vi "Modify Item Owner.vi"(8 "error in (no error)":errorcluster, 9 "New Parent Fully Qualified Name":string, 10 "UniqueName Object":refnum<class "UniqueName.lvclass">, 11 "Registry in":refnum<data-value>) -> (0 "error out":errorcluster, 1 "Modified":bool, 2 "UniqueName Object out":refnum<class "UniqueName.lvclass">, 3 "Registry":refnum<data-value>)   [LabVIEW 2013, in "UniqueName.lvlib" / "NameRegistry.lvclass"]
uses:
  NameRegistry.lvclass
  UniqueNameClass/UniqueName.lvclass
  UniquenessCriteria/UniquenessCriteria.lvclass
  UniqueNameClass/Key.ctl
  StringIncrement/StringIncrement.lvclass
  RandomStringGenerator/RandomStringGenerator.lvclass
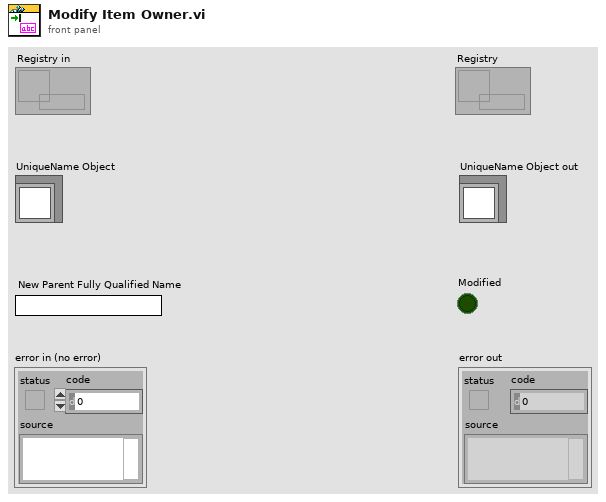
[diagram p1: front panel]
types:
  T1 = typedef "UniqueName.lvlib/UniqueName.lvclass/Key.ctl" = enum16{"Fully Qualified Name", "Unique Name", "Given Name", "Parent Fully Qualified Name", "UUID"}
  T2 = typedef "UniqueName.lvlib/UniquenessCriteria.lvclass/Criteria.ctl" = enum16{"Globally-Unique Fully Qualified Name", "Globally-Unique Name", "Universal Unique Identifier"}
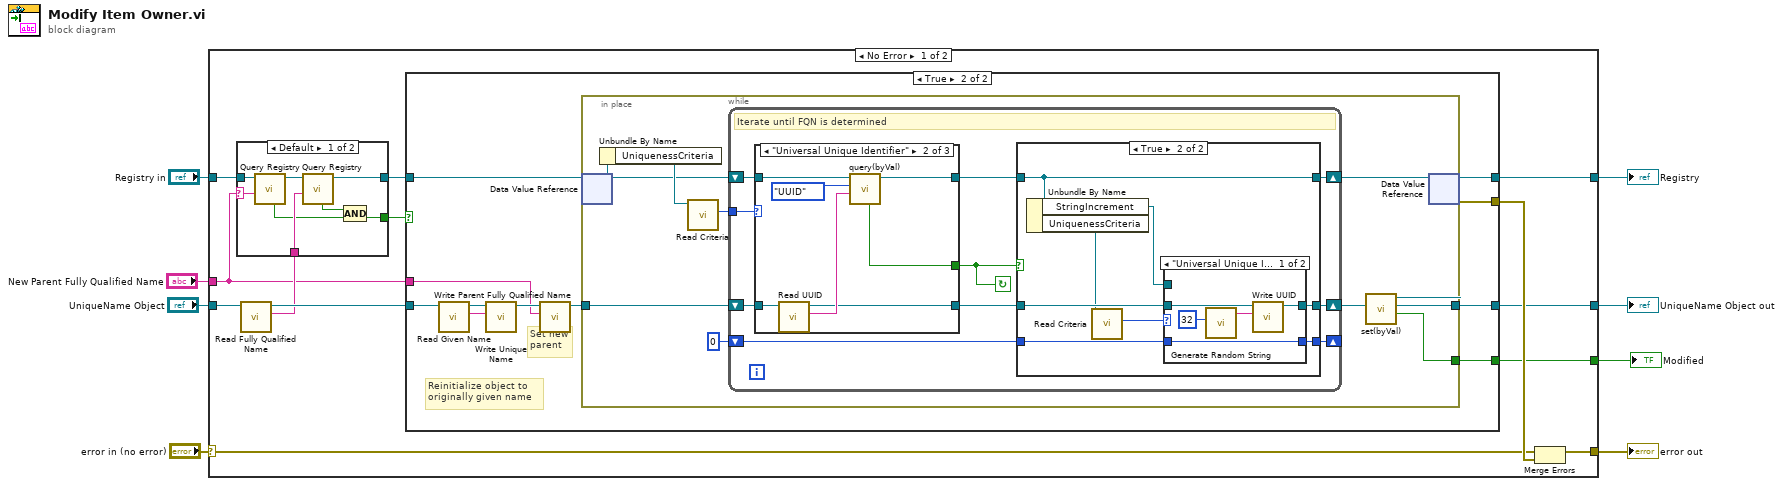
[diagram p0: block diagram]
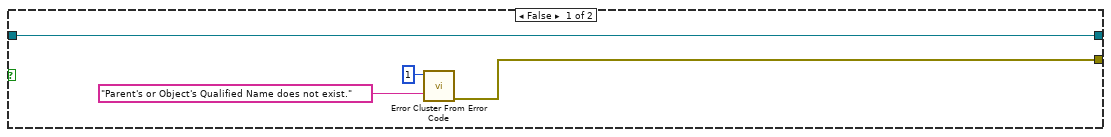
[diagram p2: hidden frame]
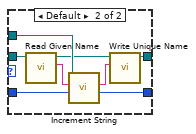
[diagram p4: hidden frame]
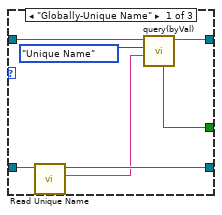
[diagram p5: hidden frame]
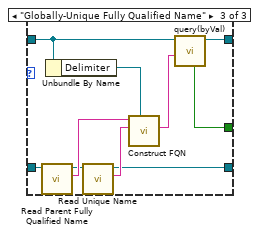
[diagram p6: hidden frame]
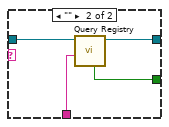
[diagram p7: hidden frame]
diagram:
  n1 = case shown="No Error" "error in (no error)" {
    selector: "error in (no error)" -> [w19 w118]
    tunnel: "Registry in" -> [w17 w119]
    tunnel: [w21 w119] -> w7
    tunnel: [w18 w118] -> w5
    tunnel: "New Parent Fully Qualified Name" -> [w10 _]
    tunnel: [w14 w117] -> w3
    tunnel: "UniqueName Object" -> [w13 w117]
    tunnel: [w9 _] -> w1
    frame No Error {
      n2 = call "Read Fully Qualified Name.vi"("UniqueName in"=w13) -> ("Fully Qualified Name"=w11:string, "UniqueName out"=w12:refnum<class "UniqueName.lvclass">)  [unwired: 9 in]
      n3 = case shown="Default" w10 {
        selector: w10 -> [w111 _]
        tunnel: w17 -> [w112 w114]
        tunnel: [w109 w116] -> w16
        tunnel: [w106 w113] -> w15
        tunnel: w11 -> [w108 w115]
        frame Default {
          n4 = call "Query Registry.vi"("Search string"=w111, "Registry in"=w112) -> ("Registry"=w110:refnum<data-value>, "found?"=w107:bool)  [unwired: 5 in, 3 out]
          n5 = call "Query Registry.vi"("Search string"=w108, "Registry in"=w110) -> ("Registry"=w109:refnum<data-value>, "found?"=w105:bool)  [unwired: 5 in, 3 out]
          n6 = Compound Arithmetic op=AND(w105, w107) -> (w106:bool)
        }
        frame "" {
          n7 = call "Query Registry.vi"("Search string"=w115, "Registry in"=w114) -> ("Registry"=w116:refnum<data-value>, "found?"=w113:bool)  [unwired: 5 in, 3 out]
        }
      }
      n8 = case shown="True" w15 {
        tunnel: [w25 w36] -> w21
        tunnel: [w23 w35] -> w20
        tunnel: w16 -> [w25 w32]
        tunnel: w10 -> [_ w33]
        tunnel: [_ w30] -> w14
        tunnel: w12 -> [_ w29]
        tunnel: [_ w26] -> w9
        frame False {
          n9 = call <vilib>:"Error Cluster From Error Code.vi"("error message (\"\")"="Parent's or Object's Qualified Name does not exist." ("error message (\"\")"), "error code (0)"=1) -> ("error out"=w23:errorcluster)  [unwired: 7 in]
        }
        frame True {
          # "Set new\nparent"
          # "Reinitialize object to\noriginally given name"
          n10 = call "Read Given Name.vi"("UniqueName in"=w29) -> ("Given Name"=w28:string, "UniqueName out"=w27:refnum<class "UniqueName.lvclass">)  [unwired: 9 in]
          n11 = call "Write Unique Name.vi"("Unique Name"=w28, "UniqueName in"=w27) -> ("UniqueName out"=w34:refnum<class "UniqueName.lvclass">)  [unwired: 9 in]
          n12 = call "Write Parent Fully Qualified Name.vi"("Parent Fully Qualified Name"=w33, "UniqueName in"=w34) -> ("UniqueName out"=w31:refnum<class "UniqueName.lvclass">)  [unwired: 9 in]
          n13 = in-place {
            in-place-border: w31 -> [w44]
            in-place-border: [w41] -> w30
            in-place-border: [w38] -> w26
            n14 = in-place-dvr #1(w32) -> (w43:refnum<class "NameRegistry.lvclass">)  [unwired: 1 out]
            n15 = Unbundle By Name(w43) -> ("UniquenessCriteria"=w46:refnum<class "UniquenessCriteria.lvclass">)
            n16 = call "Read Criteria.vi"("UniquenessCriteria in"=w46) -> ("Criteria"=w45:T2)  [unwired: 9 in, 1 out]
            n17 = while {
              tunnel: w45 -> [w56]
              shift-right: [w54] -> w42
              shift-left: w44 -> [w53]
              shift-right: [w49] -> w40
              shift-left: w43 -> [w51]
              shift-right: [w48] -> _
              shift-left: u32 0 ("Incremented Numeric") -> [w47]
              stop <- w52 continue-if-true
              # "Iterate until FQN is determined"
              n18 = case shown="\"Universal Unique Identifier\"" w56 {
                tunnel: [w84 w93 w98] -> w52
                tunnel: w53 -> [w87 w90 w102]
                tunnel: [w86 w88 w100] -> w55
                tunnel: w51 -> [w85 w94 w96]
                tunnel: [w81 w91 w97] -> w50
                frame "Globally-Unique Name" {
                  n19 = call "Read Unique Name.vi"("UniqueName in"=w87) -> ("Unique Name"=w82:string, "UniqueName out"=w86:refnum<class "UniqueName.lvclass">)  [unwired: 9 in]
                  n20 = call "query(byVal).vi"("Search string"=w82, "Search Key (FQN)"=Key."Unique Name" ("Key (FQN)"), "Instance"=w85) -> ("Instance"=w81:refnum<class "NameRegistry.lvclass">, "found?"=w84:bool)  [unwired: 5 in, 2 out]
                }
                frame "Universal Unique Identifier" {
                  n21 = call "Read UUID.vi"("UniqueName in"=w90) -> ("UUID"=w89:string, "UniqueName out"=w88:refnum<class "UniqueName.lvclass">)  [unwired: 9 in]
                  n22 = call "query(byVal).vi"("Search string"=w89, "Search Key (FQN)"=Key."UUID" ("Key (FQN)"), "Instance"=w94) -> ("Instance"=w91:refnum<class "NameRegistry.lvclass">, "found?"=w93:bool)  [unwired: 5 in, 2 out]
                }
                frame "Globally-Unique Fully Qualified Name" {
                  n23 = call "Read Parent Fully Qualified Name.vi"("UniqueName in"=w102) -> ("Parent Fully Qualified Name"=w104:string, "UniqueName out"=w101:refnum<class "UniqueName.lvclass">)  [unwired: 9 in]
                  n24 = Unbundle By Name(w96) -> ("Delimiter"=w95:refnum<class "Delimiter.lvclass">)
                  n25 = call "Read Unique Name.vi"("UniqueName in"=w101) -> ("Unique Name"=w103:string, "UniqueName out"=w100:refnum<class "UniqueName.lvclass">)  [unwired: 9 in]
                  n26 = call "Construct FQN.vi"("Delimiter"=w95, "Name"=w103, "Parent FQN"=w104) -> ("FQN"=w99:string)  [unwired: 8 in]
                  n27 = call "query(byVal).vi"("Search string"=w99, "Instance"=w96) -> ("Instance"=w97:refnum<class "NameRegistry.lvclass">, "found?"=w98:bool)  [unwired: 6 in, 2 out]
                }
              }
              n28 = case shown="True" w52 {
                tunnel: w55 -> [w59 w64]
                tunnel: [w59 w67] -> w54
                tunnel: w50 -> [w58 w66]
                tunnel: [w58 w66] -> w49
                tunnel: [w57 w63] -> w48
                tunnel: w47 -> [w57 w62]
                frame False {
                  # "Name already unique"
                }
                frame True {
                  n29 = Unbundle By Name(w66) -> ("StringIncrement"=w65:refnum<class "StringIncrement.lvclass">, "UniquenessCriteria"=w61:refnum<class "UniquenessCriteria.lvclass">)
                  n30 = call "Read Criteria.vi"("UniquenessCriteria in"=w61) -> ("Criteria"=w60:T2)  [unwired: 9 in, 1 out]
                  n31 = case shown="\"Universal Unique Identifier\"" w60 {
                    tunnel: [w71 w80] -> w67
                    tunnel: w65 -> [_ w78]
                    tunnel: w64 -> [w70 w77]
                    tunnel: [w72 w74] -> w63
                    tunnel: w62 -> [w72 w73]
                    frame "Universal Unique Identifier" {
                      n32 = call "Generate Random String.vi"("String Length (32)"=u32 32) -> ("Random String"=w69:string)  [unwired: 10 in]
                      n33 = call "Write UUID.vi"("UUID"=w69, "UniqueName in"=w70) -> ("UniqueName out"=w71:refnum<class "UniqueName.lvclass">)  [unwired: 9 in]
                    }
                    frame Default {
                      n34 = call "Read Given Name.vi"("UniqueName in"=w77) -> ("Given Name"=w76:string, "UniqueName out"=w75:refnum<class "UniqueName.lvclass">)  [unwired: 9 in]
                      n35 = call "Increment String.vi"("Numeric"=w73, "Input String"=w76, "StringIncrement"=w78) -> ("Incremented Numeric"=w74:u32, "Incremented String"=w79:string)  [unwired: 7 in]
                      n36 = call "Write Unique Name.vi"("Unique Name"=w79, "UniqueName in"=w75) -> ("UniqueName out"=w80:refnum<class "UniqueName.lvclass">)  [unwired: 9 in]
                    }
                  }
                }
              }
            }
            n37 = call "set(byVal).vi"("UniqueName in"=w42, "NameRegistry in"=w40) -> ("Replaced?"=w38:bool, "UniqueName out"=w41:refnum<class "UniqueName.lvclass">, "NameRegistry out"=w39:refnum<class "NameRegistry.lvclass">)  [unwired: 7 in]
            n38 = in-place-dvr #1(w39) -> (w36:refnum<data-value>, w35:errorcluster)
          }
        }
      }
      n39 = Merge Errors(w19, w20) -> (w18:errorcluster)
    }
    frame Error {
    }
  }
  "error out" <- w5
  "Registry" <- w7
  "UniqueName Object out" <- w3
  "Modified" <- w1
